vi "query Axis Parameter List.vi"(8 "error in (no error)":errorcluster, 11 "Interface_3D Controller in":refnum<class "Interface_3D Controller.lvclass">) -> (0 "error out":errorcluster, 1 "Valid":bool, 2 "Axis Parameter List":T1, 3 "Interface_3D Controller out":refnum<class "Interface_3D Controller.lvclass">)   [LabVIEW 2023, in "FCC 3D Controller for BS.lvlib" / "Interface_3D Controller.lvclass"]
uses:
  Interface_3D Controller.lvclass
  Type Definition/TYPE Axis Parameter List.ctl
  FCC 3D Controller for BS.lvlib
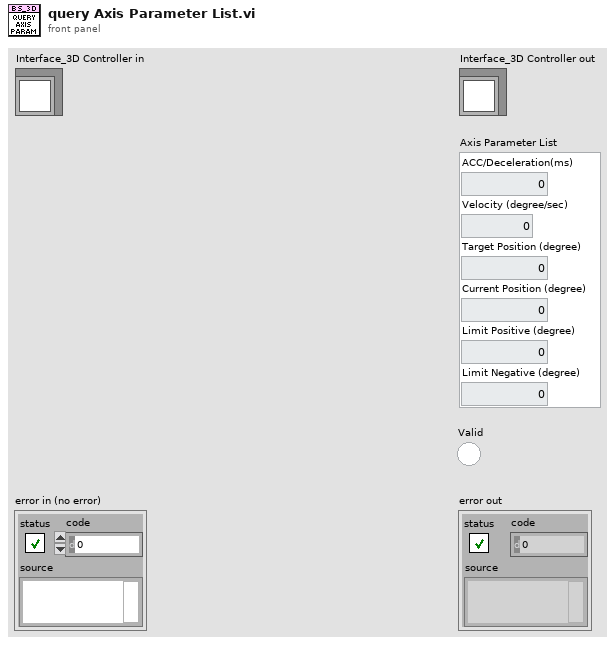
[diagram p1: front panel]
types:
  T1 = typedef "FCC 3D Controller for BS.lvlib/TYPE Axis Parameter List.ctl" = cluster{"ACC/Deceleration(ms)":dbl, "Velocity (degree/sec)":dbl, "Target Position (degree)":dbl, "Current Position (degree)":dbl, "Limit Positive (degree)":dbl, "Limit Negative (degree)":dbl}
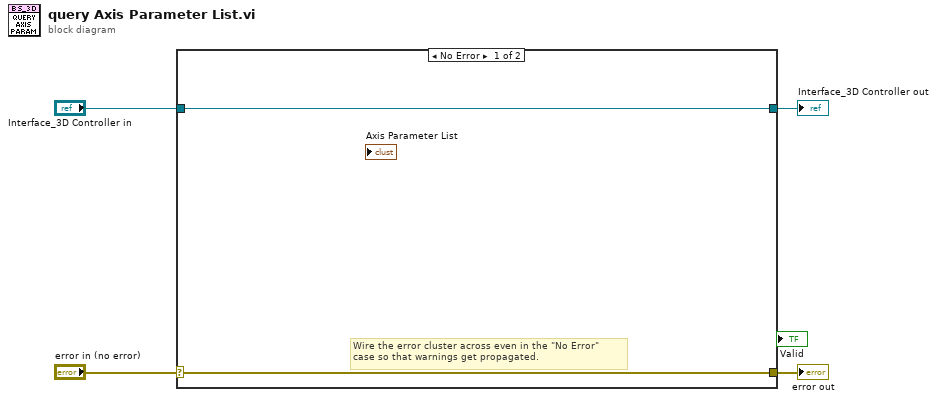
[diagram p0: block diagram]
diagram:
  n1 = case shown="No Error" "error in (no error)" {
    selector: "error in (no error)" -> [w5 w8]
    tunnel: [w5 w8] -> w3
    tunnel: [w6 w7] -> w1
    tunnel: "Interface_3D Controller in" -> [w6 w7]
    frame No Error {
      # "Wire the error cluster across even in the \"No Error\"\ncase so that warnings get propagated."
    }
    frame Error {
    }
  }
  "error out" <- w3
  "Interface_3D Controller out" <- w1
